vi "Stream to Image Files-example-v3.vi"() -> ()   [LabVIEW 2025]
doc: "The Stream to Image Files example shows how to save images to PNG files in parallel when using a grab acquisition. Images acquired from a camera are stored in a manager and each worker loop removes an image from the manager to save to disk. When the save to disk is complete, the image is added back to the manager so it can be used to copy acquired images into again. It is recommended to use the Stream to Image Files (Optimized Performance) example if your camera settings work with a ring acquisition."
uses:
  <vilib>/vision/driver/NI_Vision_Acquisition_Software.lvlib
  <resource>/objmgr/imaqdx.rc
  <vilib>/vision/driver/IMAQdx.llb/IMAQdx Buffer Number Mode.ctl
  VIs_needed/Grab Manager Mode.ctl
panel:
  out "Images Acquired Per Second":dbl
  in  "Skip Count":u32
  out "Images Behind":i32
  out "Images Saved Per Second":dbl
  in  "Number of Images":u32=30
  out "Destination Folder":path
  out "Write Speed":dbl(graph) caption="Image File Write Speed"
  in  "Camera Name":refnum<k21> caption="IMAQdx Session"
  in  "Stop":bool
  # "Overview: Demonstrates how to stream images to disk in parallel when using a ring acquisition.\nRequirements: Vision Acquisition Software\nInstructions:\n1. Select the Camera Name\n2. Run the VI\n3. Reduce the Number of Workers to see if the streaming of images can keep up with fewer workers.\n4. Increase the Skip Count if Images Behind is greater than 0."
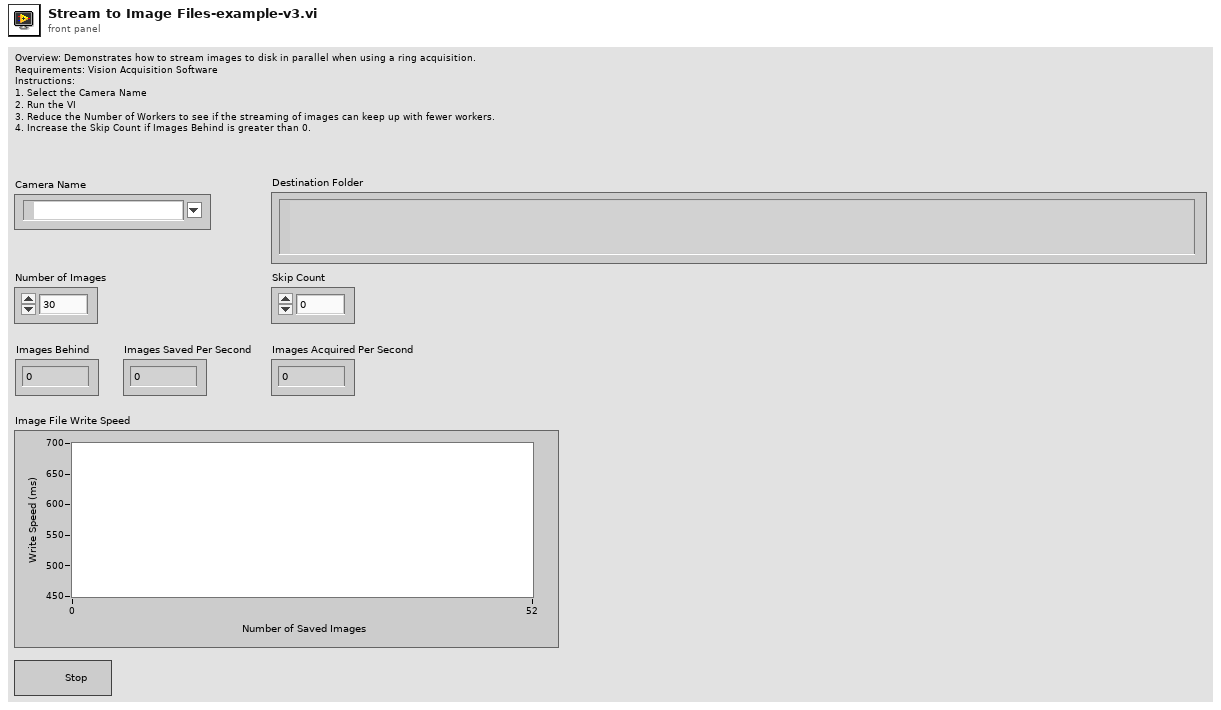
[diagram p1: front panel]
types:
  T1 = cluster{"Number of Processing Images":u32, "Image Border Size":u32}
  T2 = typedef "Grab Manager Mode.ctl" = enum16{"Create Processing Images", "Lock", "Add Acquired Image", "Get Acquired Image", "Unlock", "Dispose Processing Images"}
  T3 = typedef "IMAQdx.ctl" = refnum<k21>
  T4 = typedef "NI_Vision_Acquisition_Software.lvlib/IMAQdx Buffer Number Mode.ctl" = enum32{"Next", "Last", "Buffer Number", "Every", "Last New"}
  T5 = typedef "IMAQ Image.ctl" = refnum<image>
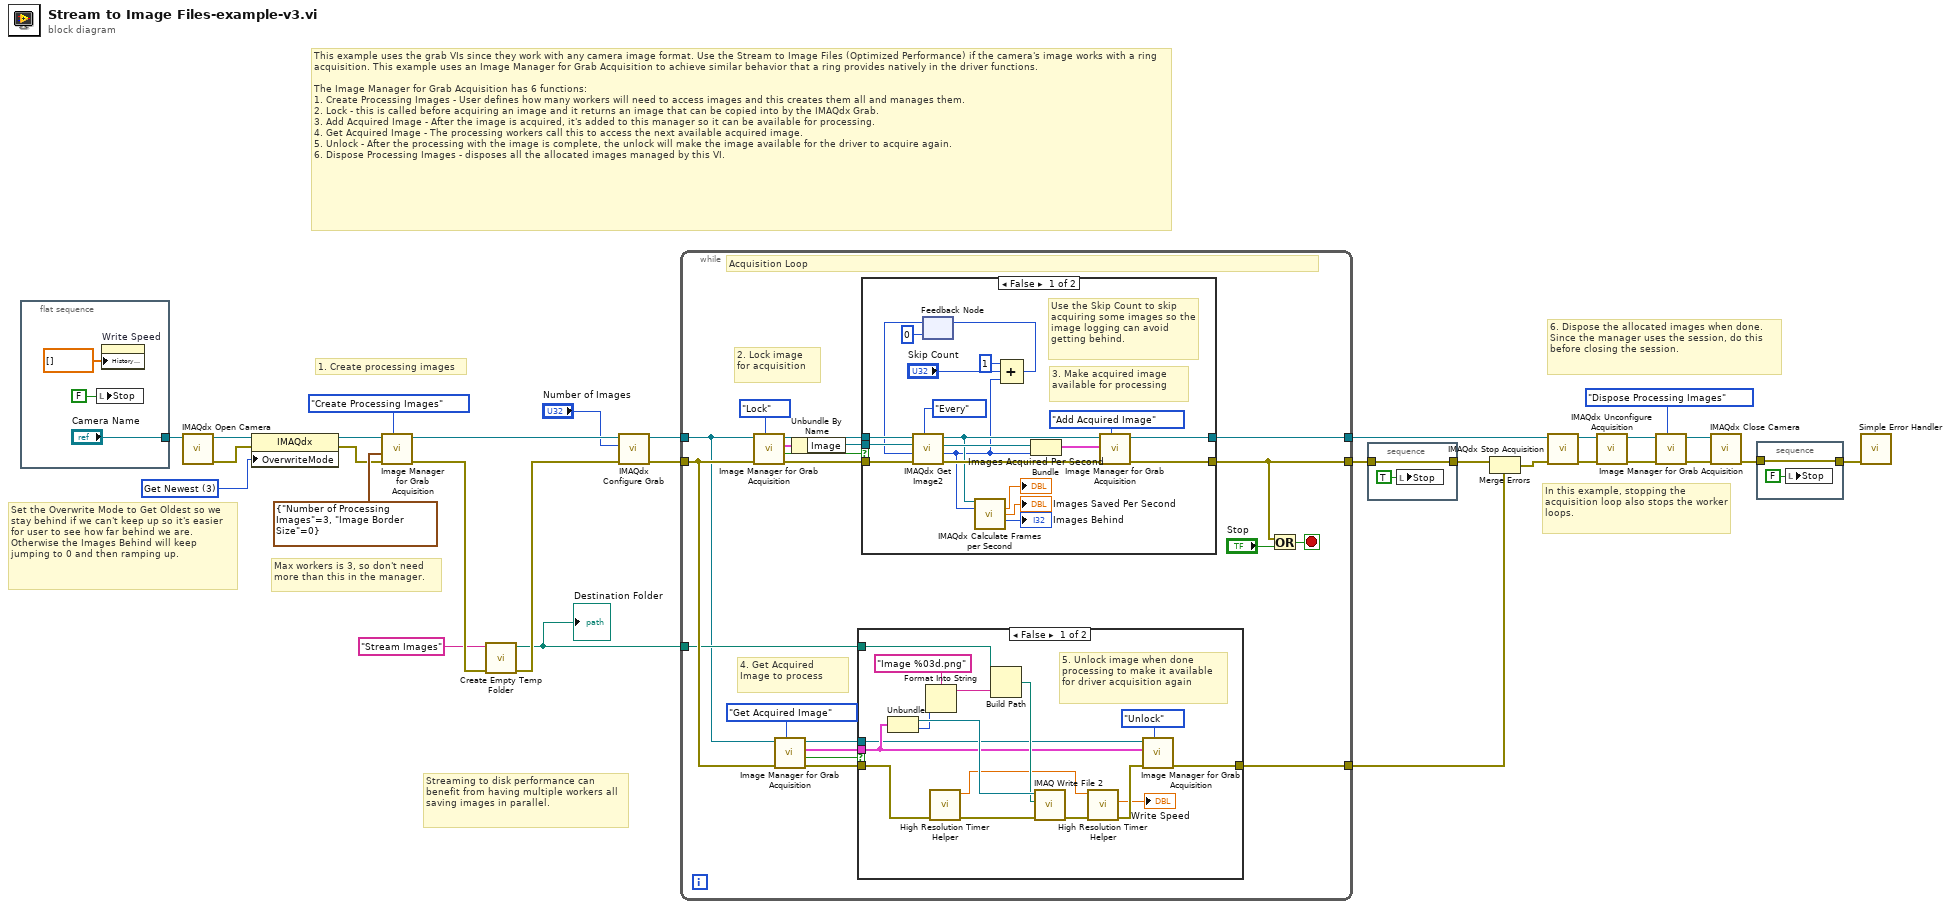
[diagram p0: block diagram]
diagram:
  w21 = u32 3 items=["Get Oldest"=0, "Fail"=2, "Get Newest"=3] ("OverwriteMode")
  # "6. Dispose the allocated images when done. Since the manager uses the session, do this before closing the session."
  # "1. Create processing images"
  # "This example uses the grab VIs since they work with any camera image format. Use the Stream to Image Files (Optimized Performance) if the camera's image works with a ring acquisition. This example uses an Image Manager for Grab Acquisition to achieve similar behavior that a ring provides natively in the driver functions.\n\nThe Image Manager for Grab Acquisition has 6 functions:\n1. Create Processing Images - User defines how many workers will need to access images and this creates them all and manages them.\n2. Lock - this is called before acquiring an image and it returns an image that can be copied into by the IMAQdx Grab.\n3. Add Acquired Image - After the image is acquired, it's added to this manager so it can be available for processing.\n4. Get Acquired Image - The processing workers call this to access the next available acquired image.\n5. Unlock - After the processing with the image is complete, the unlock will make the image available for the driver to acquire again.\n6. Dispose Processing Images - disposes all the allocated images managed by this VI."
  # "Set the Overwrite Mode to Get Oldest so we stay behind if we can't keep up so it's easier for user to see how far behind we are. Otherwise the Images Behind will keep jumping to 0 and then ramping up."
  # "Max workers is 3, so don't need more than this in the manager."
  # "In this example, stopping the acquisition loop also stops the worker loops."
  # "Streaming to disk performance can benefit from having multiple workers all saving images in parallel."
  n1 = flat-sequence {
    tunnel: ["Camera Name"] -> w30
    frame #0 {
      n2 = local write "Stop"(FALSE ("Stop")) -> ()
      n3 = property on="Write Speed" class="WFChart (strict)"("History Data"=dbl[] []) -> ()  [unwired: 2 in, 2 out]
    }
  }
  n4 = call <vilib>:"IMAQdx Open Camera.vi"("Session In"=w30) -> ("error out"=w12:errorcluster, "Session Out"=w22:T3)  [unwired: 2 in, 7 out]
  n5 = property class="IMAQdx"(reference=w22, error in=w12, "OverwriteMode"=w21) -> (reference out=w11:T3, error out=w10:errorcluster)
  n6 = call "Image Manager for Grab Acquisition.vi"("Mode"=Grab_Manager_Mode."Create Processing Images", "error in (no error)"=w10, "Init Settings"=T1 {"Number of Processing Images"=3, "Image Border Size"=0}, "Session In"=w11) -> ("error out"=w9:errorcluster, "Session Out"=w7:T3)  [unwired: 4 in, 2 out]
  n7 = call "Create Empty Temp Folder.vi"("error in (no error)"=w9, "Folder Name"="Stream Images") -> ("error out"=w6:errorcluster, "Empty Temp Folder"=w2:path)  [unwired: 8 in]
  "Destination Folder" <- w2
  n8 = call <vilib>:"IMAQdx Configure Grab.vi"("error in"=w6, "Number of Buffers"="Number of Images", "Session In"=w7) -> ("error out"=w4:errorcluster, "Session Out"=w5:T3)  [unwired: 7 in]
  n9 = while {
    tunnel: w4 -> [w42]
    tunnel: w5 -> [w40]
    tunnel: [w49] -> w26
    tunnel: [w50] -> w25
    tunnel: w2 -> [w41]
    tunnel: [w39] -> w1
    stop <- w51 stop-if-true
    # "4. Get Acquired Image to process"
    # "2. Lock image for acquisition"
    # "Acquisition Loop"
    n10 = call "Image Manager for Grab Acquisition.vi"("Mode"=Grab_Manager_Mode."Lock", "error in (no error)"=w42, "Session In"=w40) -> ("error out"=w45:errorcluster, "No Available Image"=w46:bool, "Image Settings Out"=w44:cluster{"Image":T5, "Buffer Number":u32}, "Session Out"=w47:T3)  [unwired: 5 in]
    n11 = call "Image Manager for Grab Acquisition.vi"("Mode"=Grab_Manager_Mode."Get Acquired Image", "error in (no error)"=w42, "Session In"=w40) -> ("error out"=w35:errorcluster, "No Available Image"=w37:bool, "Image Settings Out"=w36:cluster{"Image":T5, "Buffer Number":u32}, "Session Out"=w34:T3)  [unwired: 5 in]
    n12 = Unbundle By Name(w44) -> ("Image"=w43:T5)
    n13 = case shown="False" w37 {
      tunnel: w35 -> [w58 w69]
      tunnel: w36 -> [w60 _]
      tunnel: [w62 w69] -> w39
      tunnel: w41 -> [w67 _]
      tunnel: w34 -> [w59 _]
      frame False {
        # "5. Unlock image when done processing to make it available for driver acquisition again"
        n14 = Unbundle(w60) -> ("Image"=w68:T5, "Buffer Number"=w64:u32)
        n15 = Format Into String(format string="Image %03d.png", w64) -> (resulting string=w66:string)  [unwired: 2 in, 1 out]
        n16 = call "High Resolution Timer Helper.vi"("error in (no error)"=w58) -> ("error out"=w57:errorcluster, "Current Time"=w54:dbl)  [unwired: 8 in, 1 out]
        n17 = Build Path(base path=w67, name or relative path=w66) -> (appended path=w63:path)
        n18 = call-poly "IMAQ Write File 2"("error in (no error)"=w57, "File Path"=w63, "Image"=w68) -> ("error out"=w56:errorcluster)  [unwired: 7 in, 1 out]
        n19 = call "High Resolution Timer Helper.vi"("error in (no error)"=w56, "Previous Time"=w54) -> ("error out"=w55:errorcluster, "Time Difference (ms)"=→"Write Speed":dbl)  [unwired: 7 in, 1 out]
        n20 = call "Image Manager for Grab Acquisition.vi"("Mode"=Grab_Manager_Mode."Unlock", "error in (no error)"=w55, "Image Settings In"=w60, "Session In"=w59) -> ("error out"=w62:errorcluster)  [unwired: 4 in, 3 out]
      }
      frame True {
        # "No acquired images to process"
      }
    }
    n21 = case shown="False" w46 {
      tunnel: [w81 w91] -> w49
      tunnel: [w80 w90] -> w50
      tunnel: w47 -> [w89 w91]
      tunnel: w45 -> [w88 w90]
      tunnel: w43 -> [w82 _]
      frame False {
        # "3. Make acquired image available for processing"
        # "Use the Skip Count to skip acquiring some images so the image logging can avoid getting behind."
        n22 = feedback #1(u32 0) -> (w71:u32)
        n23 = call <vilib>:"IMAQdx Get Image2.vi"("Buffer Number Mode (Next)"=IMAQdx_Buffer_Number_Mode."Every", "error in"=w88, "Buffer Number In"=w71, "Image In"=w82, "Session In"=w89) -> ("error out"=w84:errorcluster, "Buffer Number Out"=w75:u32, "Image Out"=w86:T5, "Session Out"=w79:T3)  [unwired: 3 in]
        n24 = call <vilib>:"IMAQdx Calculate Frames per Second.vi"("Session In"=w79, "Buffer Number"=w75) -> ("Acquired Frames per Second"=→"Images Acquired Per Second":dbl, "Processed Frames per Second"=→"Images Saved Per Second":dbl, "Images Behind"=→"Images Behind":i32)  [unwired: 7 in, 4 out]
        n25 = Compound Arithmetic op=ADD(u32 1 ("value"), "Skip Count", w75) -> (w72:u32)
        n26 = feedback-in #1(w72) -> ()
        n27 = Bundle("Image Out"=w86, "Buffer Number Out"=w75) -> (w85:cluster{"Image Out":T5, "Buffer Number Out":u32})  [unwired: 1 in]
        n28 = call "Image Manager for Grab Acquisition.vi"("Mode"=Grab_Manager_Mode."Add Acquired Image", "error in (no error)"=w84, "Image Settings In"=w85, "Session In"=w79) -> ("error out"=w80:errorcluster, "Session Out"=w81:T3)  [unwired: 4 in, 2 out]
      }
      frame True {
        # "The Lock function already has a delay inside when no images are available to prevent loop from going too fast and starving the worker threads from getting processing time."
        # "Write to disk operation is taking longer so images aren't added back to manager. Wait until there is an available image"
      }
    }
    n29 = Or(x=w50, y="Stop") -> (x .or. y?=w51:bool)
  }
  n30 = stacked-sequence {
    tunnel: [w92] -> w24
    tunnel: w25 -> [w92]
    frame #0 {
      n31 = local write "Stop"(TRUE ("Stop")) -> ()
    }
  }
  n32 = Merge Errors(w24, w1) -> (w27:errorcluster)
  n33 = call <vilib>:"IMAQdx Stop Acquisition.vi"("error in"=w27, "Session In"=w26) -> ("error out"=w28:errorcluster, "Session Out"=w29:T3)  [unwired: 8 out]
  n34 = call <vilib>:"IMAQdx Unconfigure Acquisition.vi"("error in"=w28, "Session In"=w29) -> ("error out"=w19:errorcluster, "Session Out"=w20:T3)  [unwired: 8 out]
  n35 = call "Image Manager for Grab Acquisition.vi"("Mode"=Grab_Manager_Mode."Dispose Processing Images", "error in (no error)"=w19, "Session In"=w20) -> ("error out"=w16:errorcluster, "Session Out"=w17:T3)  [unwired: 5 in, 2 out]
  n36 = call <vilib>:"IMAQdx Close Camera.vi"("error in"=w16, "Session In"=w17) -> ("error out"=w15:errorcluster)  [unwired: 9 out]
  n37 = stacked-sequence {
    tunnel: [w94] -> w23
    tunnel: w15 -> [w94]
    frame #0 {
      n38 = local write "Stop"(FALSE ("Stop")) -> ()
    }
  }
  n39 = call <vilib>:"Simple Error Handler.vi"("error in (no error)"=w23) -> ()  [unwired: 4 in, 5 out]
